vi "Test - Insert Case.vi"(6 "Month File":string, 7 "Now":timestamp, 8 "error in":errorcluster, 9 "Inserted Entry":T1, 10 "Original Entry":T1, 11 "Case Folder":path) -> (0 "error out":errorcluster, 1 "Running Text":string, 2 "Reread Text":string, 3 "Pieces Text":string, 4 "Month File Changed?":bool, 5 "Insert Error Code":i32)   [LabVIEW 2026]
doc: "Test support for Test Insert Entry.vi. Runs Insert Entry.vi once on the data in Case Folder and reports what it did as text, formatted by Test - Format Entries.vi so it can be compared with expected text. The insert's own error is returned as Insert Error Code and cleared; any other error is passed on. After the insert the stores are initialized again from Case Folder, so Reread Text comes from the month files: each saved piece read back with Read Entry by its ID and Start Time (so from the month of its own start), followed by the original ID read back at the original Start Time (none when it was deleted).\n\nInputs: Case Folder; Original Entry; Inserted Entry; Now; Month File (the original's month file name, compared before and after); error in.\nOutputs: Pieces Text; Reread Text; Running Text; Insert Error Code; Month File Changed?; error out.\n\nGenerated by: Claude"
uses:
  Storage/Time Entry Store/Time Entry Store.lvclass
  Storage/Rows/Time Entry.ctl
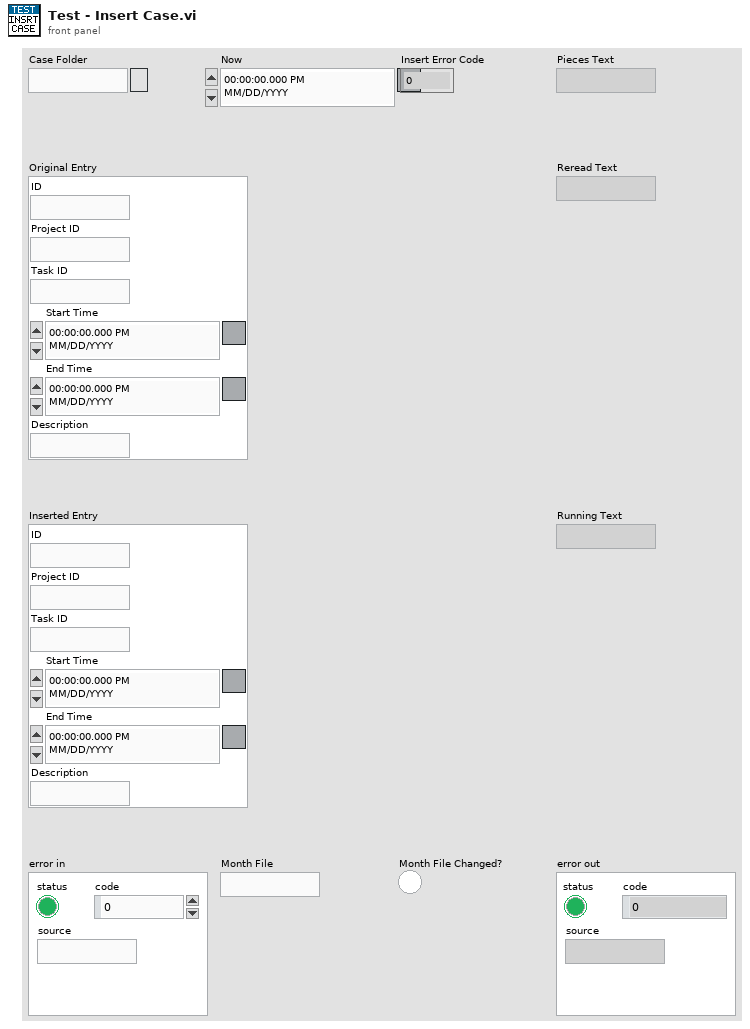
[diagram p1: front panel]
types:
  T1 = typedef "Time Entry.ctl" = cluster{"ID":string, "Project ID":string, "Task ID":string, "Start Time":timestamp, "End Time":timestamp, "Description":string}
  T2 = typedef "Time Entry List.ctl" = T1[]
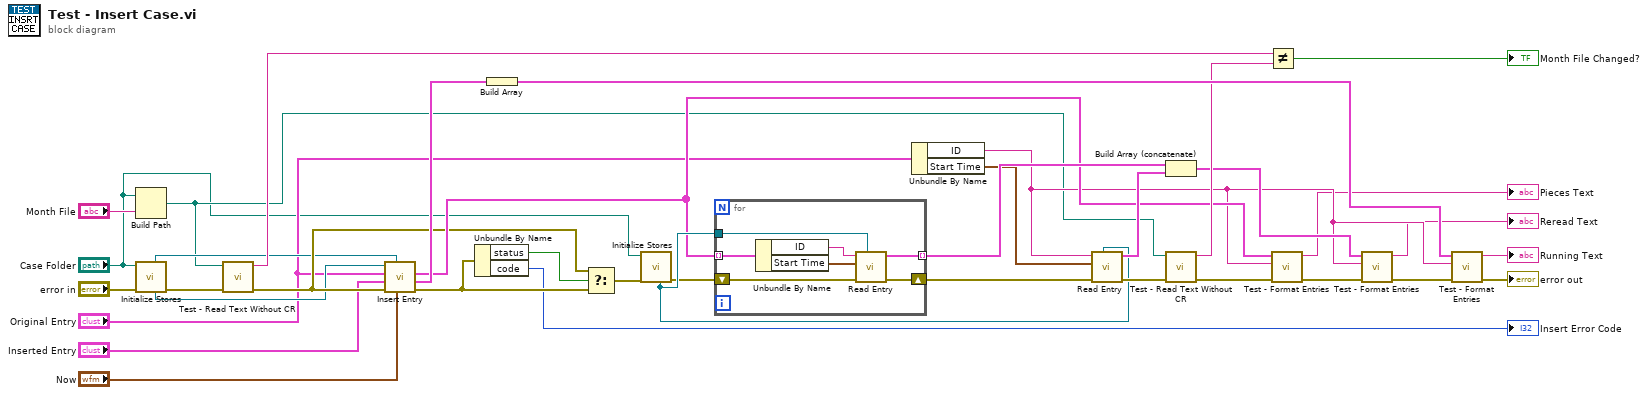
[diagram p0: block diagram]
diagram:
  n1 = Build Path(base path="Case Folder", name or relative path="Month File") -> (appended path=w13:path)
  n2 = call "Initialize Stores.vi"("error in"="error in", "Data Folder"="Case Folder") -> ("error out"=w16:errorcluster, "Time Entry Store out"=w17:refnum<class "Time Entry Store.lvclass">, "Project Store out"=w18:refnum<class "Project Store.lvclass">)  [unwired: 5 in, 2 out]
  n3 = call "Test - Read Text Without CR.vi"("error in (no error)"=w16, "File"=w13) -> ("error out"=w19:errorcluster, "Text"=w20:string)  [unwired: 8 in]
  n4 = call "Insert Entry.vi"("Now"="Now", "Project Store in"=w18, "error in"=w19, "Inserted Entry"="Inserted Entry", "Original Entry"="Original Entry", "Time Entry Store in"=w17) -> ("error out"=w23:errorcluster, "Running Entry"=w22:T1, "Pieces"=w21:T2)  [unwired: 1 in, 2 out]
  n5 = Unbundle By Name(w23) -> ("status"=w24:bool, "code"=→"Insert Error Code":i32)
  n6 = Build Array(w22) -> (w35:T1[])
  n7 = Select(t=w19, s=w24, f=w23) -> (s? t:f=w25:errorcluster)
  n8 = call "Initialize Stores.vi"("error in"=w25, "Data Folder"="Case Folder") -> ("error out"=w26:errorcluster, "Time Entry Store out"=w27:refnum<class "Time Entry Store.lvclass">)  [unwired: 5 in, 3 out]
  n9 = for {
    tunnel: w21 -> [w38] mode=indexing
    tunnel: w27 -> [w39]
    shift-right: [w41] -> w28
    shift-left: w26 -> [w40]
    tunnel: [w44] -> w29 mode=indexing
    n10 = Unbundle By Name(w38) -> ("ID"=w42:string, "Start Time"=w43:timestamp)
    n11 = call-dynamic "Read Entry.vi"("Time Entry Store in"=w39, "error in (no error)"=w40, "Start Time"=w43, "ID"=w42) -> ("error out"=w41:errorcluster, "Time Entry"=w44:T1)  [unwired: 4 in, 2 out]
  }
  n12 = Unbundle By Name("Original Entry") -> ("ID"=w14:string, "Start Time"=w15:timestamp)
  n13 = call-dynamic "Read Entry.vi"("Time Entry Store in"=w27, "error in (no error)"=w28, "Start Time"=w15, "ID"=w14) -> ("error out"=w31:errorcluster, "Time Entry"=w30:T1)  [unwired: 4 in, 2 out]
  n14 = Build Array (concatenate)(w29, w30) -> (w32:T1[])
  n15 = call "Test - Read Text Without CR.vi"("error in (no error)"=w31, "File"=w13) -> ("error out"=w33:errorcluster, "Text"=w34:string)  [unwired: 8 in]
  n16 = Not Equal?(x=w20, y=w34) -> (x != y?=→"Month File Changed?":bool)
  n17 = call "Test - Format Entries.vi"("error in"=w33, "Original ID"=w14, "Entries"=w21) -> ("error out"=w36:errorcluster, "Text"=→"Pieces Text":string)  [unwired: 7 in]
  n18 = call "Test - Format Entries.vi"("error in"=w36, "Original ID"=w14, "Entries"=w32) -> ("error out"=w37:errorcluster, "Text"=→"Reread Text":string)  [unwired: 7 in]
  n19 = call "Test - Format Entries.vi"("error in"=w37, "Original ID"=w14, "Entries"=w35) -> ("error out"=→"error out":errorcluster, "Text"=→"Running Text":string)  [unwired: 7 in]
